vi "Init Socket.vi"(8 "error in (no error)":errorcluster caption="에러 입력(에러 없음)", 9 "Queue Ref":T1, 10 "연결 ID":refnum<k5>, 11 "TCP Socket 입력":refnum<class "TCP Socket.lvclass">) -> (0 "error out":errorcluster caption="에러 출력", 3 "TCP Socket 출력":refnum<class "TCP Socket.lvclass">)   [LabVIEW 2023, in "TCP Socket.lvclass"]
uses:
  TCP Socket.lvclass
  TCP Socket.lvclass/TCP Socket.ctl
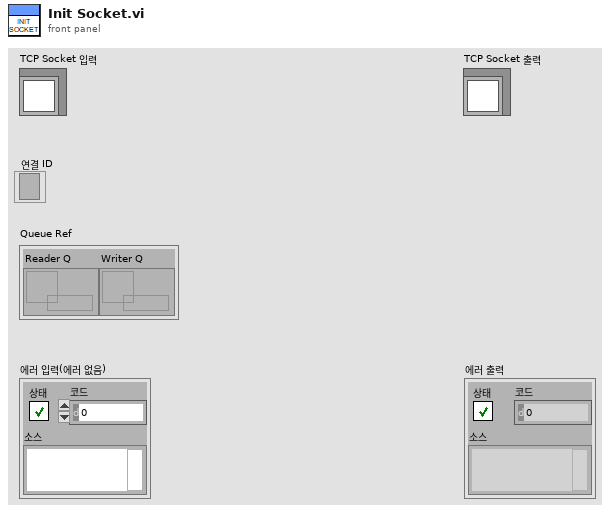
[diagram p1: front panel]
types:
  T1 = cluster{"Reader Q":refnum<queue>, "Writer Q":refnum<queue>}
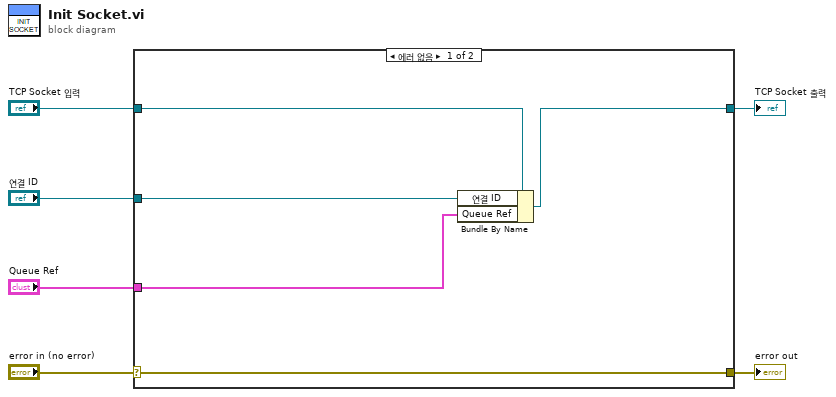
[diagram p0: block diagram]
diagram:
  n1 = case shown="에러 없음" "error in (no error)" {
    selector: "error in (no error)" -> [w11 w13]
    tunnel: [w11 w13] -> w5
    tunnel: [w9 w12] -> w3
    tunnel: "TCP Socket 입력" -> [w10 w12]
    tunnel: "연결 ID" -> [w8 _]
    tunnel: "Queue Ref" -> [w7 _]
    frame No Error {
      n2 = Bundle By Name(cluster=w10, "연결 ID"=w8, "Queue Ref"=w7) -> (w9:refnum<class "TCP Socket.lvclass">)
    }
    frame Error {
    }
  }
  "error out" <- w5
  "TCP Socket 출력" <- w3
